vi "VIH HelpGen - HTML - Extract Template Codes - Menu Help.vi"(11 "HTML in":string) -> (0 "ProductInfo Template":string, 2 "Table Templates":T1, 3 "HTML out":string)   [LabVIEW 2014]
doc: "::: VI Helpeks :::\nCopyright (c) 2000-2026 Konstantin Shifershteyn. All rights reserved."
uses:
  _VIH HelpGen.llb/VIH HelpGen Typedef - Table Templates Cluster - Menu Help.ctl
panel:
  # "VI Helpeks\nCopyright (c) 2012-2026 Konstantin Shifershteyn"
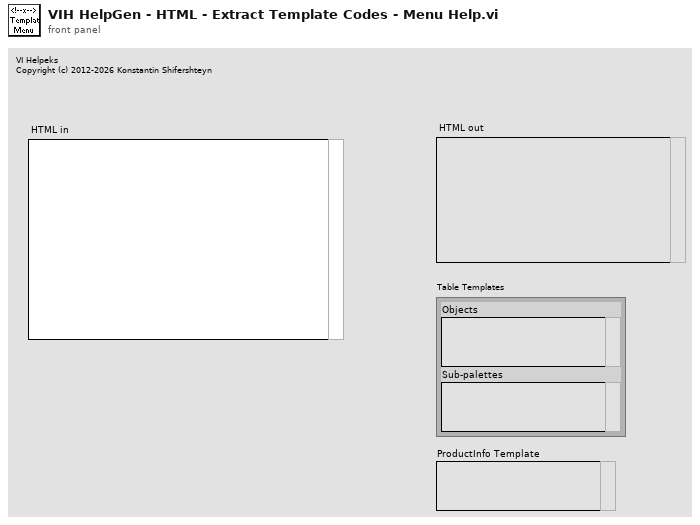
[diagram p1: front panel]
types:
  T1 = typedef "VIH HelpGen Typedef - Table Templates Cluster - Menu Help.ctl" = cluster{"Objects":string, "Sub-palettes":string}
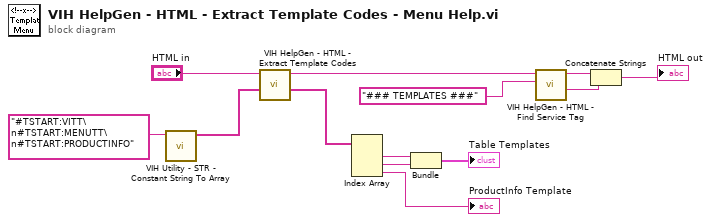
[diagram p0: block diagram]
diagram:
  n1 = call "VIH Utility - STR - Constant String To Array.vi"("String in"="#TSTART:VITT\n#TSTART:MENUTT\n#TSTART:PRODUCTINFO") -> ("Array out"=w8:string[])  [unwired: 10 in]
  n2 = call "VIH HelpGen - HTML - Extract Template Codes.vi"("Tag names"=w8, "HTML in"="HTML in") -> ("Templates"=w7:string[], "HTML out"=w6:string)  [unwired: 8 in]
  n3 = Index Array(array=w7) -> (element #1=w12:string, element #2=w11:string, element #3=→"ProductInfo Template":string)  [unwired: 3 in]
  n4 = Bundle("String"=w12, "String"=w11) -> (→"Table Templates":cluster{"String":string, "String":string})  [unwired: 1 in]
  n5 = call "VIH HelpGen - HTML - Find Service Tag.vi"("Tag name"="### TEMPLATES ###", "HTML in"=w6) -> ("After"=w3:string, "Before"=w4:string)  [unwired: 6 in, 2 out]
  n6 = Concatenate Strings(w4, w3) -> (→"HTML out":string)
